vi "GetKeyboardState Wrapper Template.vi"(11 "error in":errorcluster) -> (4 "key state":u8[](array[numeric]), 6 "return value":i32, 15 "error out":errorcluster)   [LabVIEW 2020]
doc: "Reads the key state of the CALLING thread through user32.dll GetKeyboardState (stdcall, called in LabVIEW's UI thread): one byte per virtual-key code, bit 0x80 set while the key is down, bit 0x01 the toggle state. Windows keeps this state per thread and updates it only when the thread retrieves input from the real input queue - posted messages leave it alone. Running in the UI thread, this is the state LabVIEW's panels read for the modifier keys (GetKeyState). return value is the Win32 BOOL: non-zero on success, 0 on failure. When error in carries an error the DLL is not called. Generated by scripts\\Build Win32 Wrappers.vi - do not edit by hand, rebuild it."
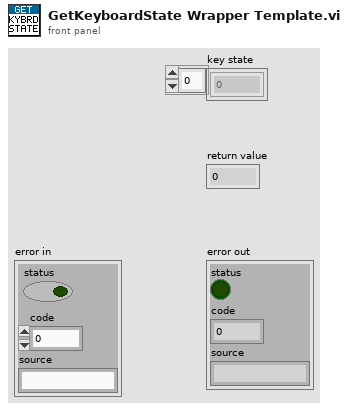
[diagram p1: front panel]
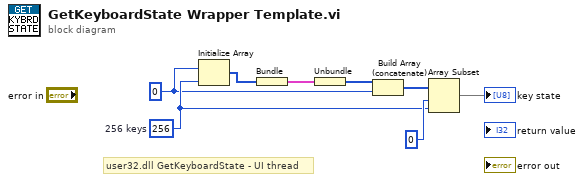
[diagram p0: block diagram]
diagram:
  w3 = 256  # 256 keys
  w2 = u8 0
  # "user32.dll GetKeyboardState - UI thread"
  n1 = Initialize Array(w2, w3) -> (w5:u8[])
  n2 = Bundle(w5) -> (w6:cluster{u8[]})  [unwired: 1 in]
  n3 = Unbundle(w6) -> (w7:u8[])
  n4 = Build Array (concatenate)(w7, w2) -> (w8:u8[])
  n5 = Array Subset(array=w8, index=0, length=w3) -> (→"key state":u8[])
